vi "TEST ManagerUI.vi"() -> ()   [LabVIEW 2021, in "Channel.lvlib" / "ChannelsManager.lvlib"]
uses:
  Channel/ChannelsManager/ChannelsManager.lvlib
  Channel/ChannelsManager/ChannelsManager/ChannelsManager.lvclass
  Channel/Channel_class/Channel.lvclass
  Channel.lvlib
panel:
  out "error out 2":errorcluster={"status"=TRUE, "code"=7, "source"="NI_LVConfig.lvlib:Load.vi"}
  in  "Config File":path=path "C:/Users/averna/Documents/LV Gym DEMO/Factory Pattern/Channels/Files/Test.ini"
  out "error out":errorcluster={"status"=TRUE, "code"=7, "source"="NI_LVConfig.lvlib:Load.vi"}
  in  "Plugins Folder":path=path "C:/Users/averna/Documents/LV Gym DEMO/Factory Pattern"
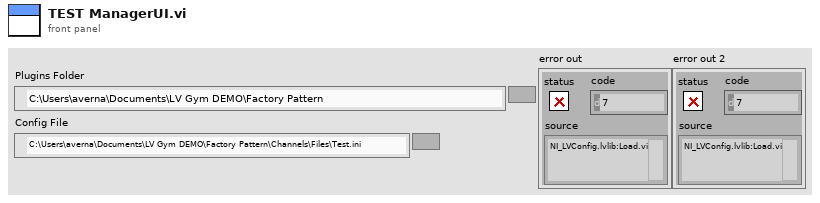
[diagram p1: front panel]
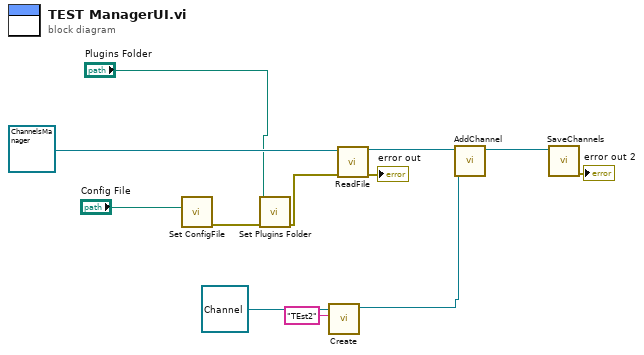
[diagram p0: block diagram]
diagram:
  n1 = call "Set ConfigFile.vi"("Plugins Folder"="Config File") -> ("error out"=w8:errorcluster)  [unwired: 10 in]
  n2 = call "Set Plugins Folder.vi"("error in (no error)"=w8, "Config File"="Plugins Folder") -> ("error out"=w7:errorcluster)  [unwired: 9 in]
  n3 = call-dynamic "Create.vi"("Name"="TEst2", "object in"=refnum<class "Channel.lvclass"> refnum ("Channel.lvlib:Channel")) -> ("object out"=w4:refnum<class "Channel.lvclass">)  [unwired: 8 in, 1 out]
  n4 = call-dynamic "ReadFile.vi"("error in (no error)"=w7, "object in"=refnum<class "ChannelsManager.lvclass"> refnum ("ChannelsManager.lvlib:ChannelsManager")) -> ("error out"=→"error out":errorcluster, "object out"=w11:refnum<class "ChannelsManager.lvclass">)  [unwired: 8 in]
  n5 = call-dynamic "AddChannel.vi"("Channel"=w4, "object in"=w11) -> ("object out"=w10:refnum<class "ChannelsManager.lvclass">)  [unwired: 8 in, 1 out]
  n6 = call "SaveChannels.vi"("object in"=w10) -> ("error out"=→"error out 2":errorcluster)  [unwired: 9 in, 1 out]
